vi "ASDE Peak Region Data Pass Formation VI.vi"(4 "S#":i32, 5 "A New folder":string, 6 "T (ms)":string="3.12", 7 "I (pA)":string="3.12", 8 "error in":errorcluster, 9 "Signal P":string="3.12", 10 "N #":string="3.12", 11 "Filename":path) -> (0 "error out":errorcluster, 3 "PSX Pass":path)   [LabVIEW 2018]
panel:
  out "取り除かれたパス 2":path
  out "取り除かれたパス":path
  out "PS? 3":bool caption="既存するファイルまたはフォルダ?"
  out "PS? 2":bool caption="既存するファイルまたはフォルダ?"
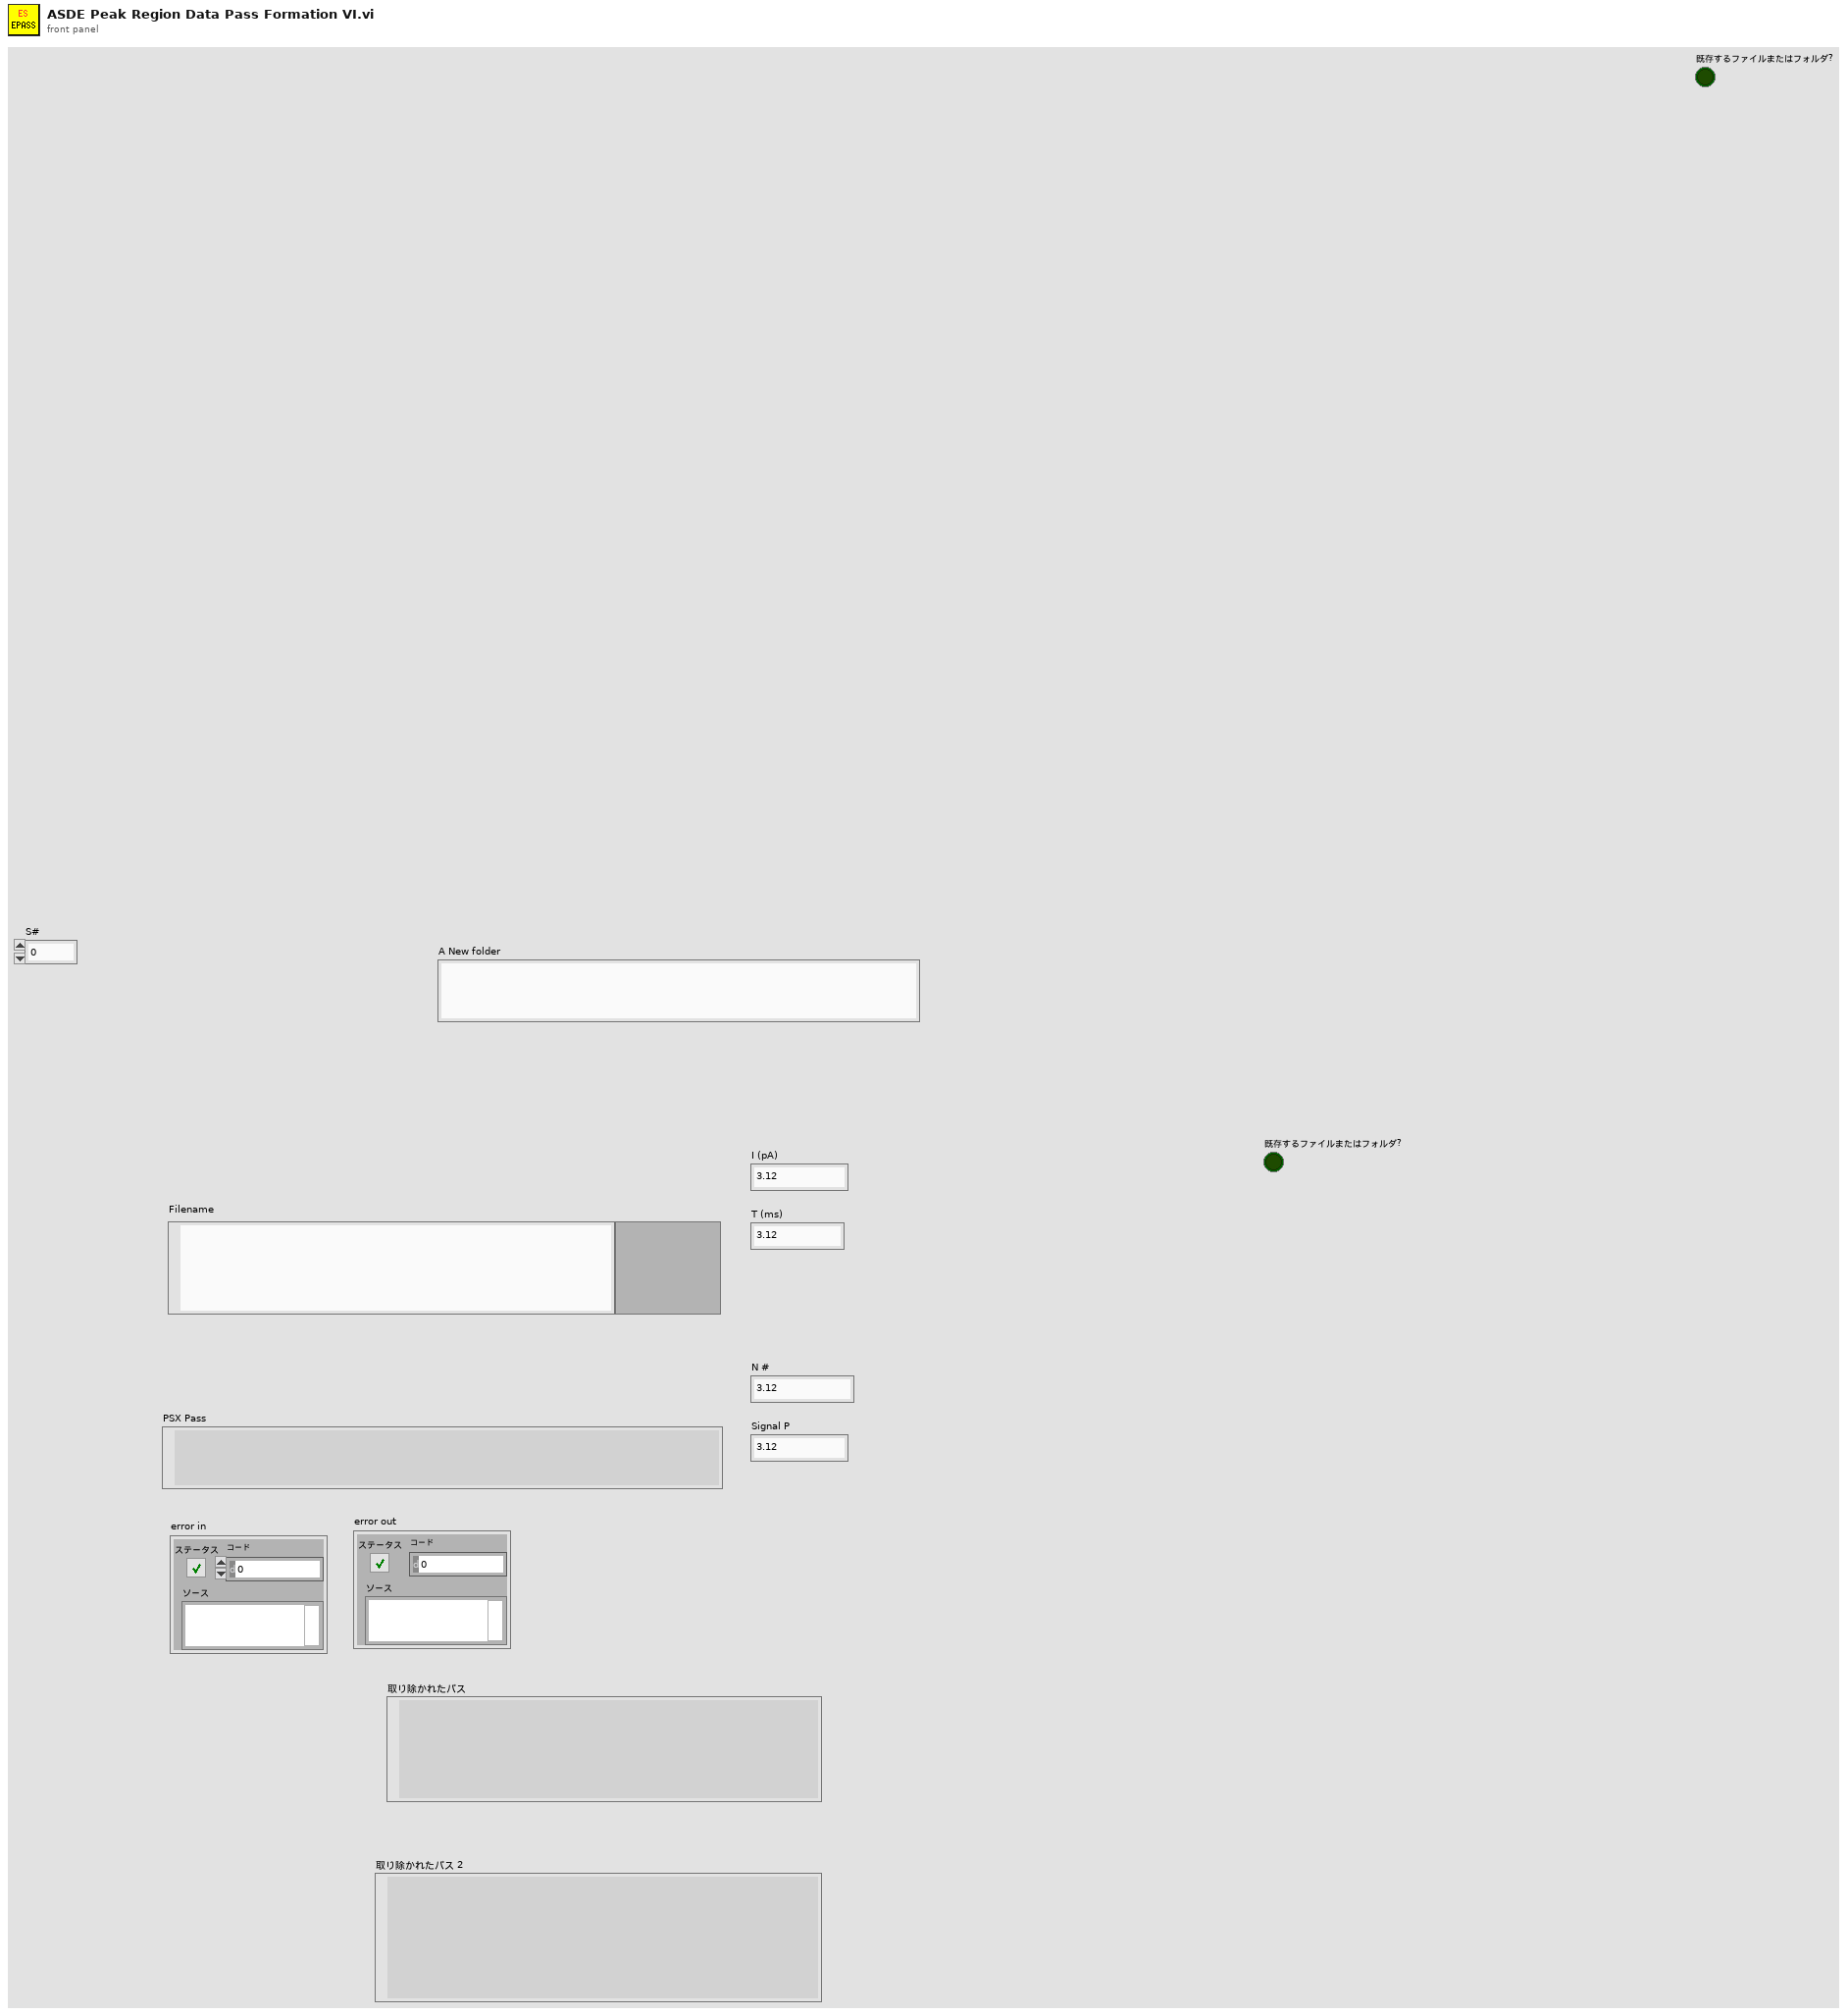
[diagram p1: front panel]
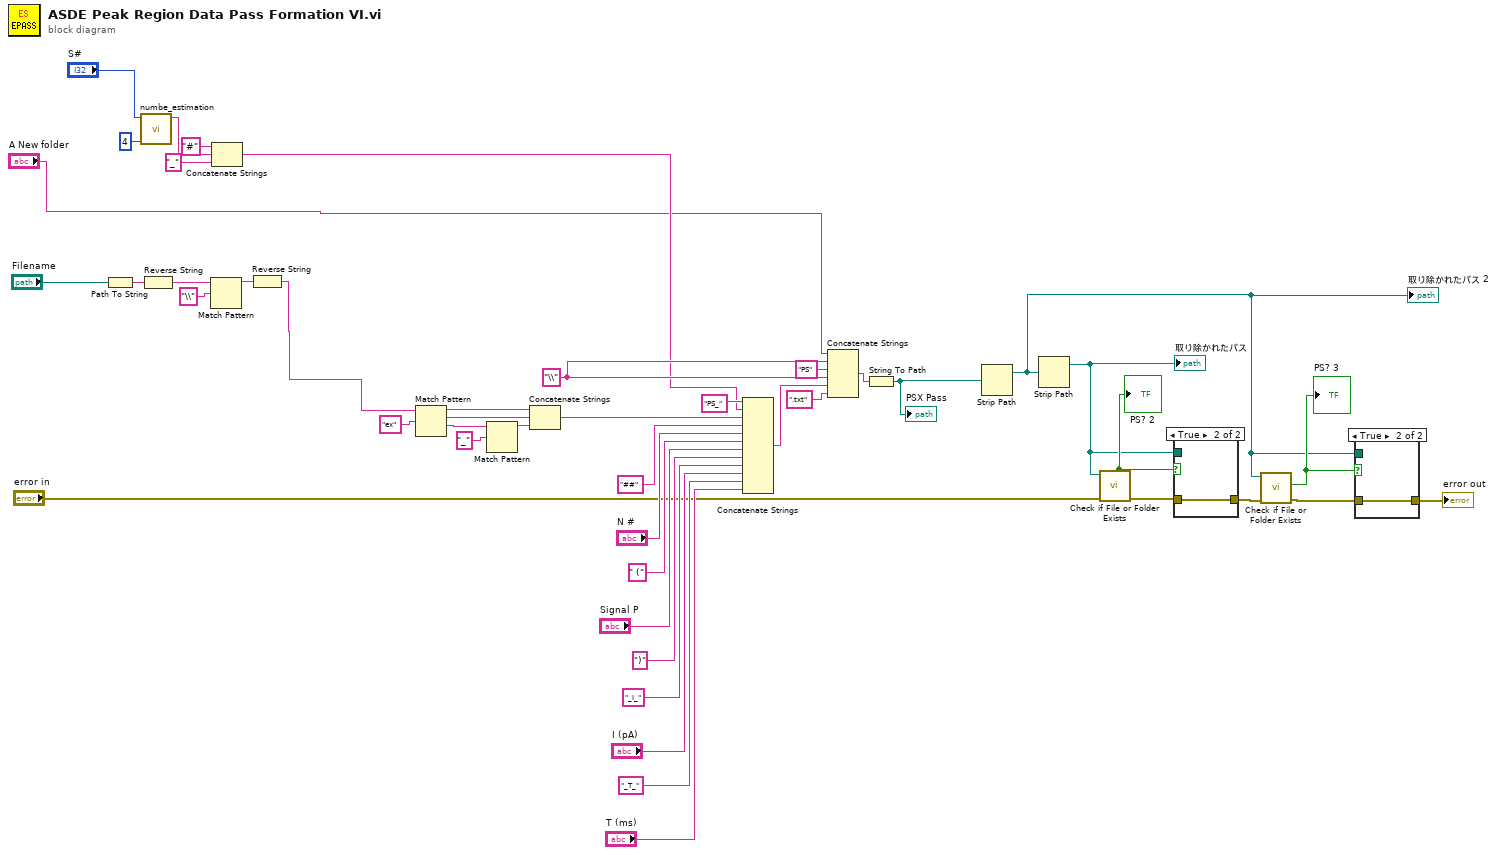
[diagram p0: block diagram]
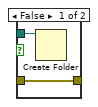
[diagram p2: hidden frame]
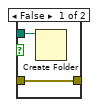
[diagram p3: hidden frame]
diagram:
  w10 = "\\" ("検索文字列")
  n1 = Path To String(path="Filename") -> (string=w42:string)
  n2 = call "numbe_estimation.vi"("桁数"=4, "数値"="S#") -> ("数値文字列"=w6:string)  [unwired: 9 in]
  n3 = Reverse String(1:w42) -> (0:w44:string)
  n4 = Match Pattern(string=w44, regular expression="\\" ("検索文字列")) -> (before substring=w43:string)  [unwired: 1 in, 3 out]
  n5 = Concatenate Strings("#" ("文字列"), w6, "_" ("文字列")) -> (w2:string)
  n6 = Reverse String(1:w43) -> (0:w36:string)
  n7 = Match Pattern(string=w36, regular expression="ex" ("正規表現")) -> (before substring=w32:string, match substring=w31:string, after substring=w33:string)  [unwired: 1 in, 1 out]
  n8 = Match Pattern(string=w33, regular expression="_" ("正規表現")) -> (before substring=w30:string)  [unwired: 1 in, 3 out]
  n9 = Concatenate Strings(w32, w31, w30) -> (w25:string)
  n10 = Concatenate Strings("PS_" ("文字列"), w2, w25, "##" ("文字列"), "N #", " (" ("文字列"), "Signal P", ")" ("文字列"), "_I_" ("文字列"), "I (pA)", "_T_" ("文字列"), "T (ms)") -> (w29:string)
  n11 = Concatenate Strings("A New folder", w10, "PS" ("文字列"), w10, w29, ".txt" ("連結文字列")) -> (w27:string)
  n12 = String To Path(string=w27) -> (path=w26:path)
  "PSX Pass" <- w26
  n13 = Strip Path(path=w26) -> (stripped path=w13:path)  [unwired: 1 out]
  "取り除かれたパス 2" <- w13
  n14 = Strip Path(path=w13) -> (stripped path=w18:path)  [unwired: 1 out]
  "取り除かれたパス" <- w18
  n15 = call <vilib>:"Check if File or Folder Exists.vi"("error in (no error)"="error in", "path"=w18) -> ("error out"=w11:errorcluster, "file or folder exists?"=w19:bool)  [unwired: 7 in, 1 out]
  "PS? 2" <- w19
  n16 = case shown="True" w19 {
    tunnel: w18 -> [w47 _]
    tunnel: w11 -> [w46 w48]
    tunnel: [w46 w48] -> w16
    frame False {
      n17 = Create Folder(path (use dialog)=w47) -> ()  [unwired: 2 in, 3 out]
    }
    frame True {
    }
  }
  n18 = call <vilib>:"Check if File or Folder Exists.vi"("error in (no error)"=w16, "path"=w13) -> ("error out"=w15:errorcluster, "file or folder exists?"=w17:bool)  [unwired: 7 in, 1 out]
  "PS? 3" <- w17
  n19 = case shown="True" w17 {
    tunnel: w13 -> [w50 _]
    tunnel: w15 -> [w49 w51]
    tunnel: [w49 w51] -> w14
    frame False {
      n20 = Create Folder(path (use dialog)=w50) -> ()  [unwired: 2 in, 3 out]
    }
    frame True {
    }
  }
  "error out" <- w14
